vi "Test U8 Publisher.vi"() -> ()   [LabVIEW 2021]
uses:
  ChannelCommon/typedef/Direction.ctl
  CIF_Iceoryx_PCAP_Universal.lvclass
  Iceorxy Utilities/Typedef/PCAP Config.ctl
  ChannelCommon/typedef/New FIFO Config.ctl
  ChannelCommon/typedef/FIFO Flags.ctl
  Iceorxy Utilities/Typedef/PCAP Linktype.ctl
  ChannelCommon/typedef/TimeStamps.ctl
  ChannelCommon/ChannelCommon.lvlib
  Iceorxy Utilities/Iceoryx Channel Utilities.lvlib
panel:
  in  "stop":bool
  out "timed out?":bool
  out "error out":errorcluster
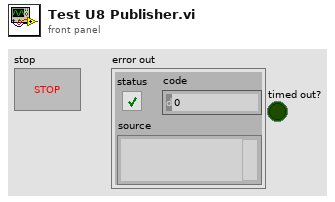
[diagram p1: front panel]
types:
  T1 = typedef "Iceoryx Channel Utilities.lvlib/PCAP Config.ctl" = cluster{"New FIFO Config":T2, "Linktype":T4, "Linktype Override":u32, "Type Name Override":string}
  T2 = typedef "ChannelCommon.lvlib/New FIFO Config.ctl" = cluster{"Max Bytes/Msg":u64, "Max Msg/FIFO":u64, "FIFO Flags":T3, "Best Effort Subscribers":u32, "Backpressure Subscribers":u32}
  T3 = typedef "ChannelCommon.lvlib/FIFO Flags.ctl" = cluster{"Backpressure":bool, "Extended Config":bool}
  T4 = typedef "Iceoryx Channel Utilities.lvlib/PCAP Linktype.ctl" = u32
  T5 = typedef "ChannelCommon.lvlib/Direction.ctl" = enum8{"Publisher", "Subscriber"}
  T6 = typedef "ChannelCommon.lvlib/TimeStamps.ctl" = cluster{"ClockID":u8, "T0":i64, "T_Out":i64}
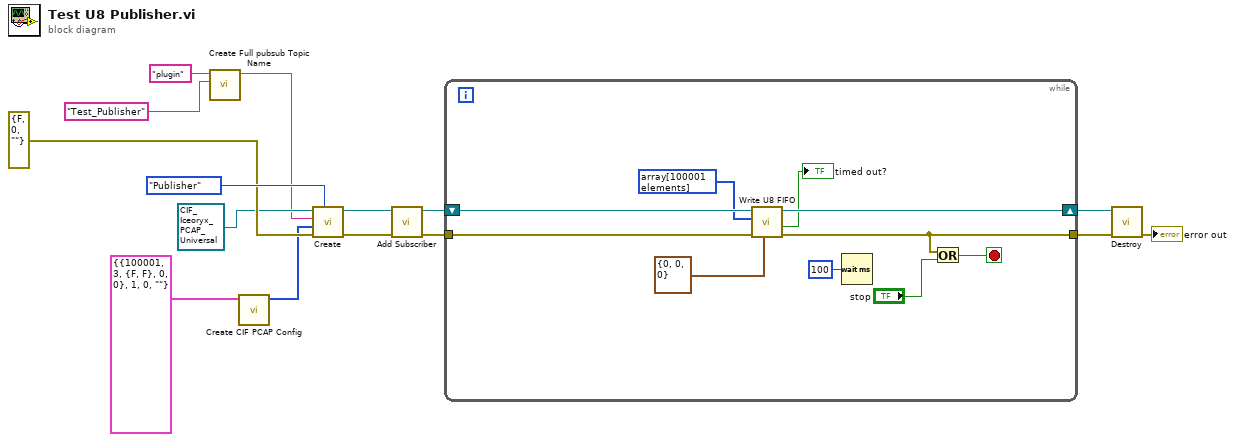
[diagram p0: block diagram]
diagram:
  n1 = call "Create Full pubsub Topic Name.vi"("Topic"="Test_Publisher" ("Name"), "Plugin name"="plugin") -> ("Full Topic"=w5:string)  [unwired: 8 in, 1 out]
  n2 = call "Create CIF PCAP Config.vi"("PCAP FIFO Config"=T1 {"New FIFO Config"={"Max Bytes/Msg"=100001, "Max Msg/FIFO"=3, "FIFO Flags"={"Backpressure"=FALSE, "Extended Config"=FALSE}, "Best Effort Subscribers"=0, "Backpressure Subscribers"=0}, "Linktype"=1, "Linktype Override"=0, "Type Name Override"=""}) -> ("Flattened PCAP FIFO Config"=w8:u8[])  [unwired: 10 in]
  n3 = call-dynamic "Create.vi"("Direction"=Direction."Publisher", "error in (no error)"=errorcluster {"status"=FALSE, "code"=0, "source"=""} ("error out"), "Custom Config Data"=w8, "Name"=w5, "CIFFIFO in"=refnum<class "CIF_Iceoryx_PCAP_Universal.lvclass"> refnum ("CIF_CIPC_Fifo_U8.lvclass")) -> ("error out"=w3:errorcluster, "CIFFIFO out"=w4:refnum<class "CIF_Iceoryx_PCAP_Universal.lvclass">)  [unwired: 5 in]
  n4 = call-dynamic "Add Subscriber.vi"("error in (no error)"=w3, "CIF_CIPC_Chn in"=w4) -> ("error out"=w1:errorcluster, "CIF_CIPC_Chn out"=w2:refnum<class "CIF_Iceoryx_PCAP_Universal.lvclass">)  [unwired: 7 in, 1 out]
  n5 = while {
    shift-right: [w22] -> w13
    shift-left: w2 -> [w24]
    tunnel: w1 -> [w23]
    tunnel: [w18] -> w12
    stop <- w16 stop-if-true
    n6 = call-dynamic "Write U8 FIFO.vi"("FIFO Timestamps"=T6 {"ClockID"=0, "T0"=0, "T_Out"=0}, "error in (no error)"=w23, "Data in"=u8[] array[100001 elements] ("U8 Data"), "CIFFIFO in"=w24) -> ("error out"=w18:errorcluster, "timed out?"=→"timed out?":bool, "CIFFIFO out"=w22:refnum<class "CIF_Iceoryx_PCAP_Universal.lvclass">)  [unwired: 4 in, 1 out]
    n7 = Wait (ms)(milliseconds to wait=u32 100) -> ()  [unwired: 1 out]
    n8 = Or(x=w18, y="stop") -> (x .or. y?=w16:bool)
  }
  n9 = call-dynamic "Destroy.vi"("error in (no error)"=w12, "Icoryx_PCAP in"=w13) -> ("error out"=→"error out":errorcluster)  [unwired: 8 in, 1 out]
